vi "TCP Server Set Modified Data.vi"(8 "error in (no error)":errorcluster, 10 "Data in":T1, 11 "RefNum":refnum<class "JKI TCP Server.lvclass">) -> (0 "error out":errorcluster, 3 "dup RefNum":refnum<class "JKI TCP Server.lvclass">)   [LabVIEW 2020, in "JKI TCP Server.lvclass"]
doc: "Sets the GOOP data structure and releases mutex"
uses:
  JKI TCP Server.lvclass
  _Data Structures/TCP Server Data.ctl
  _Data Structures/TCP Server Listener Info Cluster.ctl
  _Data Structures/TCP Server Connection Info Cluster.ctl
  _Data Structures/TCP Server Handler RefNum.ctl
  _Data Structures/TCP Server Object Data Core Task Enum.ctl
  JKI TCP Server.lvclass/JKI TCP Server.ctl
panel:
  # "OpenGOOP Set Modified Data.vi\n\nSets the GOOP data structure and releases mutex\n\nCopyright (C) 2002, 2003 Jim Kring jim@jimkring.com\n\nPlease visit http://www.OpenG.org to learn about the\nOpen Source LabVIEW software movement.\n\nThis library is free software; you can redistribute it and/or\nmodify it under the terms of the GNU Lesser General Public\nLicense as published by the Free Software Foundation; either\nversion 2.1 of the License, or (at your option) any later version.\nThis library is distributed in the hope that it will be useful,\nbut WITHOUT ANY WARRANTY; without even the implied warranty of\nMERCHANTABILITY or FITNESS FOR A PARTICULAR PURPOSE. See the GNU\nLesser General Public License for more details.\nYou should have received a copy of the GNU Lesser General Public\nLicense along with this library; if not, write to the Free Software\nFoundation, Inc., 59 Temple Place, Suite 330, Boston, MA 02111-1307 USA"
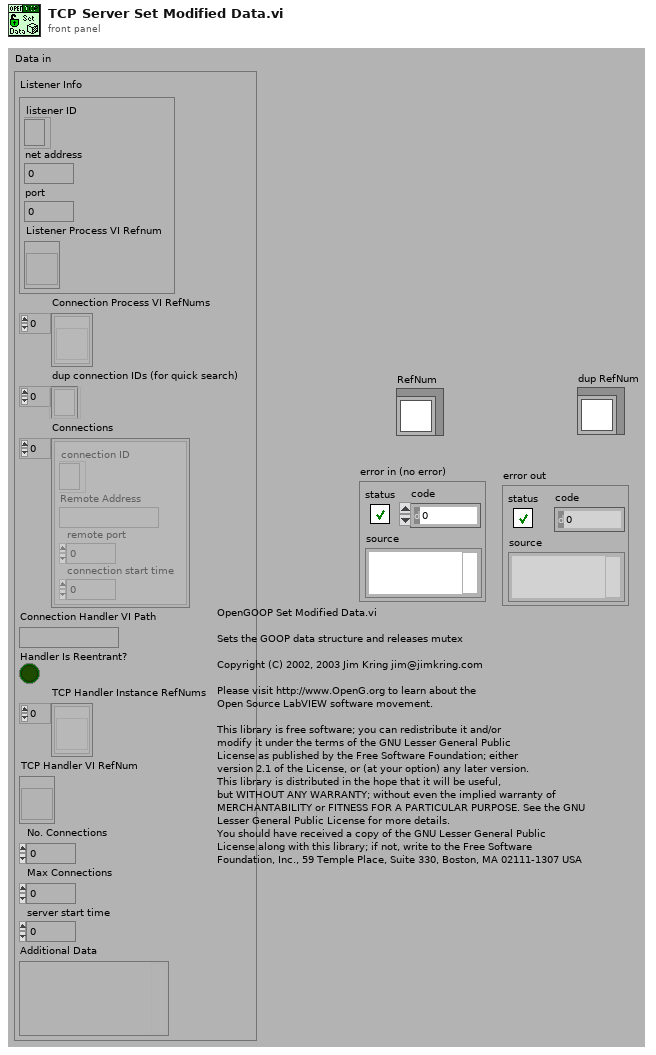
[diagram p1: front panel]
types:
  T1 = typedef "JKI TCP Server.lvclass/TCP Server Data.ctl" = cluster{"Listener Info":T2, "Connection Process VI RefNums":refnum<vi>[], "dup connection IDs (for quick search)":refnum<k5>[], "Connections":T3[], "Connection Handler VI Path":path, "Handler Is Reentrant?":bool, "TCP Handler Instance RefNums":T4[], "TCP Handler VI RefNum":T4, "No. Connections":u32, "Max Connections":u32, "server start time":u32, "Additional Data":variant}
  T2 = typedef "JKI TCP Server.lvclass/TCP Server Listener Info Cluster.ctl" = cluster{"listener ID":refnum<k5>, "net address":u32, "port":u16, "Listener Process VI Refnum":refnum<vi>}
  T3 = typedef "JKI TCP Server.lvclass/TCP Server Connection Info Cluster.ctl" = cluster{"connection ID":refnum<k5>, "Remote Address":string, "remote port":u16, "connection start time":u32}
  T4 = typedef "JKI TCP Server.lvclass/TCP Server Handler RefNum.ctl" = refnum<vi>
  T5 = typedef "JKI TCP Server.lvclass/TCP Server Object Data Core Task Enum.ctl" = enum16{"read", "write", "init"}
  T6 = typedef "Semaphore RefNum" = refnum<k1>
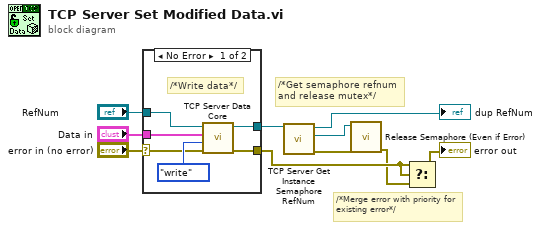
[diagram p0: block diagram]
diagram:
  # "/*Merge error with priority for existing error*/"
  # "/*Get semaphore refnum and release mutex*/"
  n1 = case shown="No Error" "error in (no error)" {
    selector: "error in (no error)" -> [w15 w18]
    tunnel: [w12 w18] -> w6
    tunnel: "Data in" -> [w14 _]
    tunnel: "RefNum" -> [w13 w17]
    tunnel: [w11 w17] -> w7
    frame No Error {
      # "/*Write data*/"
      n2 = call "TCP Server Data Core.vi"("error in (no error)"=w15, "task (read)"=TCP_Server_Object_Data_Core_Task_Enum."write", "Data in"=w14, "Refnum"=w13) -> ("error out"=w12:errorcluster, "dup Refnum"=w11:refnum<class "JKI TCP Server.lvclass">)  [unwired: 5 in, 1 out]
    }
    frame Error {
    }
  }
  n3 = call "TCP Server Get Instance Semaphore RefNum.vi"("RefNum"=w7) -> ("error in (no error)"=w4:errorcluster, "semaphore"=w1:T6, "dup RefNum"=→"dup RefNum":refnum<class "JKI TCP Server.lvclass">)  [unwired: 8 in]
  n4 = call "Release Semaphore (Even if Error).vi"("error in (no error)"=w4, "semaphore"=w1) -> ("error out"=w3:errorcluster)  [unwired: 8 in, 1 out]
  n5 = Select(t=w6, s=w6, f=w3) -> (s? t:f=→"error out":errorcluster)
